vi "test Get Parameters.vi"(8 "error in":errorcluster, 11 "TestCase in":refnum<class "Scripting.lvclass">) -> (0 "error out":errorcluster, 3 "TestCase out":refnum<class "Scripting.lvclass">)   [LabVIEW 2020, in "Scripting.lvclass"]
uses:
  Scripting.lvclass
  <vilib>/addons/_JKI Toolkits/VI Tester/TestCase.llb/TestCase.lvclass
  Scripting/AIM/Constants.vi
  Scripting/AIM/AIM ARINC 429 Scripting.lvlib
  <vilib>/NI/NI VeriStand Encoding and Decoding/Encoding.ctl
  <vilib>/NI/NI VeriStand Encoding and Decoding/Encoding and Decoding.lvlib
  Shared/Parameter Definition.ctl
  <vilib>/NI VeriStand/Custom Device Tools/Custom Device Utility Library/Custom Device Utility Library.lvlib
  Shared/Label Properties.ctl
  <vilib>/NI VeriStand/Custom Device API/Custom Device API.lvlib
  Shared/Label.ctl
  Shared/Direction.ctl
  Shared/VS Channel Definition for Parameter.ctl
  Shared/Transfer Type.ctl
  Shared/VS Channels Definition for Label.ctl
  <vilib>/NI VeriStand/Custom Device Tools/Custom Device Utility Library/NI VeriStand - Search for Item by GUID.vi
  Shared/Transfer Speed.ctl
  C:/Program Files (x86)/National Instruments/LabVIEW 2020/vi.lib/addons/_JKI Toolkits/VI Tester/TestCase.llb/TestCase.lvclass
  C:/git/ni/niveristand-aim-arinc429-custom-device/Source/Custom Device Support/Tests/Unit/Scripting/Scripting.lvclass
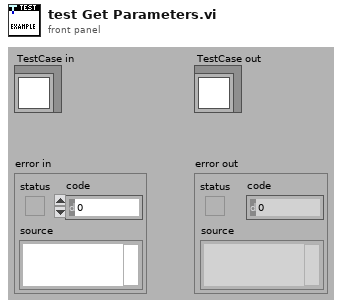
[diagram p1: front panel]
types:
  T1 = typedef "Transfer Speed.ctl" = enum16{"LO (12.5 kb/s)", "HI (100 kb/s)"}
  T2 = typedef "VS Channels Definition for Label.ctl" = cluster{"label (Dec)":u32, "parameters":T3[], "SDI value":u8, "SDI enabled":bool, "transfer type":T6, "create timestamp":bool, "transmit period":u32}
  T3 = typedef "VS Channel Definition for Parameter.ctl" = cluster{"name":string, "unit":string, "Parameter":T4}
  T4 = typedef "Parameter Definition.ctl" = cluster{"start index":i32, "size":i32, "encoding":T5, "signed":bool, "scale multiplier":dbl, "scale offset":dbl, "default value":dbl}
  T5 = typedef "Encoding and Decoding.lvlib/Encoding.ctl" = enum16{"BNR", "BCD", "Discrete"}
  T6 = typedef "Transfer Type.ctl" = enum16{"Scheduled", "Acyclic", "Block", "Strobe"}
  T7 = typedef "Direction.ctl" = enum16{"Rx", "Tx"}
  T8 = typedef "Label Properties.ctl" = cluster{"label (Dec)":T9, "SDI value":u8, "SDI enabled":bool}
  T9 = typedef "Label.ctl" = u8
  T10 = typedef "Custom Device API.lvlib/Custom Device Item Ref.ctl" = u64
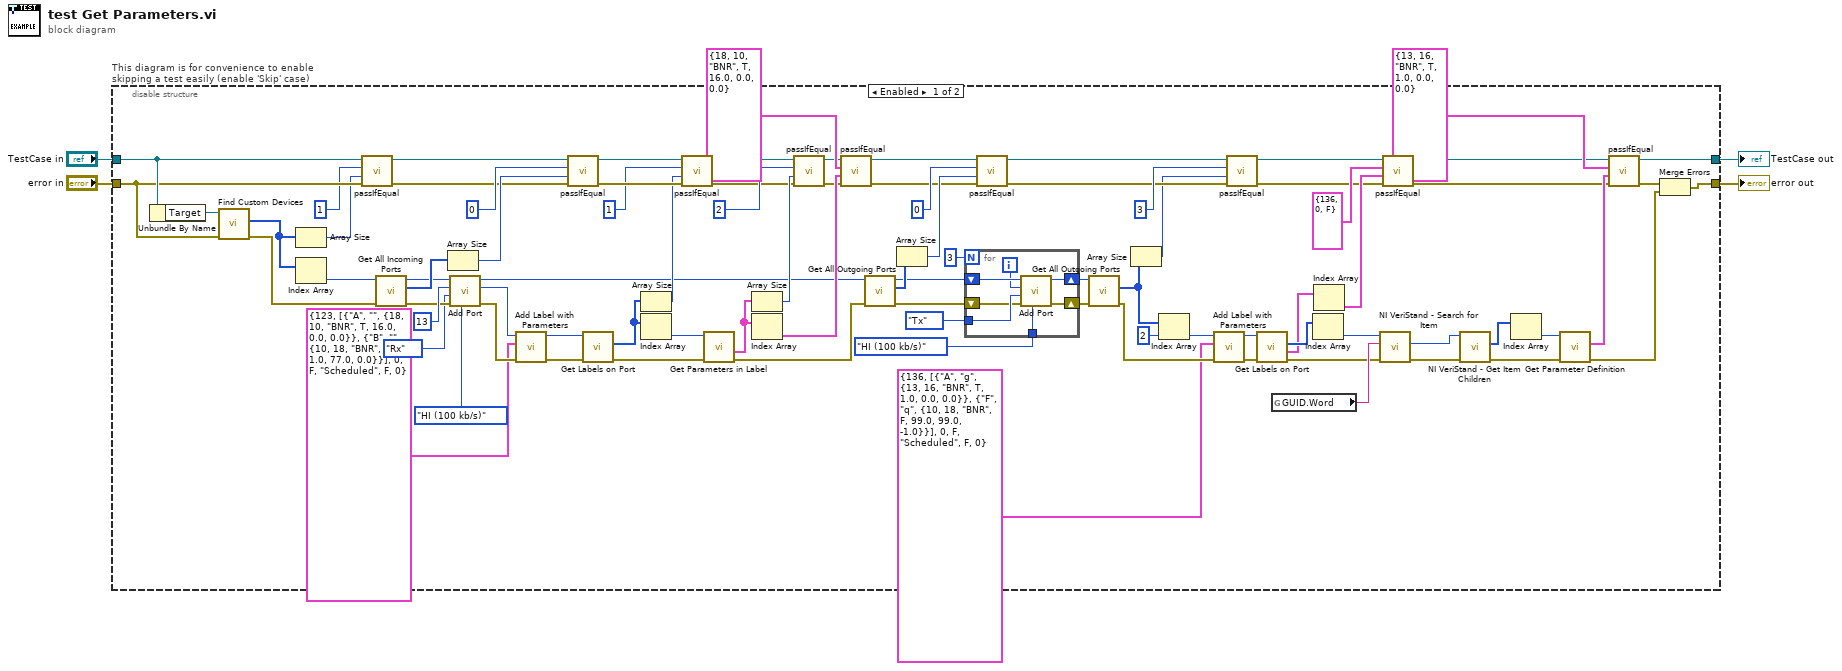
[diagram p0: block diagram]
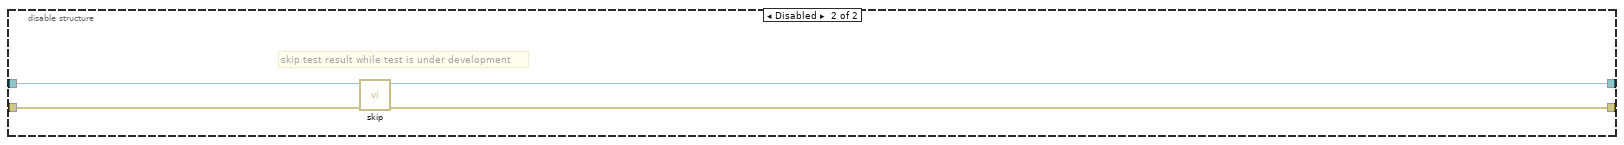
[diagram p2: hidden frame]
diagram:
  n1 = disable-structure "This diagram is for convenience to enable skipping a test easily (enable 'Skip' case)" shown="Enabled" {
    disable-tunnel: "TestCase in" -> [w87 w101]
    disable-tunnel: [w68 w99] -> w1
    disable-tunnel: [w70 w100] -> w3
    disable-tunnel: "error in" -> [w86 w98]
    frame Enabled {
      n2 = Unbundle By Name(w87) -> ("Target"=w89:refnum<k24>)
      n3 = call "Find Custom Devices.vi"("error in"=w86, "target in"=w89) -> ("error out"=w78:errorcluster, "AIM ARINC 429 custom devices"=w35:u64[])  [unwired: 7 in, 1 out]
      n4 = Array Size(array=w35) -> (size(s)=w84:i32)
      n5 = Index Array(array=w35) -> (element=w88:u64)  [unwired: 1 in]
      n6 = call-dynamic "passIfEqual.vi"("error in (no error)"=w86, "y"=w84, "x"=1 ("size(s)"), "TestCase in"=w87) -> ("error out"=w79:errorcluster, "TestCase out"=w80:refnum<class "Scripting.lvclass">)  [unwired: 6 in]
      n7 = call "Get All Incoming Ports.vi"("error in"=w78, "AIM ARINC 429 custom device in"=w88) -> ("error out"=w31:errorcluster, "incoming ports"=w83:T10[], "AIM ARINC 429 custom device out"=w34:T10)  [unwired: 7 in]
      n8 = Array Size(array=w83) -> (size(s)=w81:i32)
      n9 = call "Add Port.vi"("speed"=Transfer_Speed."HI (100 kb/s)", "error in"=w31, "direction"=Direction."Rx", "port number"=u16 13, "AIM ARINC 429 custom device in"=w34) -> ("error out"=w28:errorcluster, "port"=w29:T10, "AIM ARINC 429 custom device out"=w33:T10)  [unwired: 4 in]
      n10 = call "Add Label with Parameters.vi"("error in"=w28, "label"=T2 {"label (Dec)"=123, "parameters"=[{"name"="A", "unit"="", "Parameter"={"start index"=18, "size"=10, "encoding"=enum."BNR", "signed"=TRUE, "scale multiplier"=16.0, "scale offset"=0.0, "default value"=0.0}}, {"name"="B", "unit"="", "Parameter"={"start index"=10, "size"=18, "encoding"=enum."BNR", "signed"=FALSE, "scale multiplier"=1.0, "scale offset"=77.0, "default value"=0.0}}], "SDI value"=0, "SDI enabled"=FALSE, "transfer type"=enum."Scheduled", "create timestamp"=FALSE, "transmit period"=0}, "port ref"=w29) -> ("error out"=w25:errorcluster, "port ref out"=w26:T10)  [unwired: 7 in]
      n11 = call-dynamic "passIfEqual.vi"("error in (no error)"=w79, "y"=w81, "x"=0 ("size(s)"), "TestCase in"=w80) -> ("error out"=w62:errorcluster, "TestCase out"=w63:refnum<class "Scripting.lvclass">)  [unwired: 6 in]
      n12 = call "Get Labels on Port.vi"("error in"=w25, "port in"=w26) -> ("error out"=w50:errorcluster, "labels"=w51:T10[])  [unwired: 6 in, 2 out]
      n13 = Array Size(array=w51) -> (size(s)=w59:i32)
      n14 = Index Array(array=w51) -> (element=w61:T10)  [unwired: 1 in]
      n15 = call-dynamic "passIfEqual.vi"("error in (no error)"=w62, "y"=w59, "x"=1 ("size(s)"), "TestCase in"=w63) -> ("error out"=w54:errorcluster, "TestCase out"=w55:refnum<class "Scripting.lvclass">)  [unwired: 6 in]
      n16 = call "Get Parameters in Label.vi"("error in"=w50, "label in"=w61) -> ("error out"=w65:errorcluster, "parameter definitions"=w58:T4[])  [unwired: 6 in, 2 out]
      n17 = Array Size(array=w58) -> (size(s)=w56:i32)
      n18 = Index Array(array=w58) -> (element=w64:T4)  [unwired: 1 in]
      n19 = call-dynamic "passIfEqual.vi"("error in (no error)"=w54, "y"=w56, "x"=2 ("size(s)"), "TestCase in"=w55) -> ("error out"=w52:errorcluster, "TestCase out"=w53:refnum<class "Scripting.lvclass">)  [unwired: 6 in]
      n20 = call-dynamic "passIfEqual.vi"("error in (no error)"=w52, "y"=w64, "x"=T4 {"start index"=18, "size"=10, "encoding"=enum."BNR", "signed"=TRUE, "scale multiplier"=16.0, "scale offset"=0.0, "default value"=0.0} ("parameter definition"), "TestCase in"=w53) -> ("error out"=w74:errorcluster, "TestCase out"=w75:refnum<class "Scripting.lvclass">)  [unwired: 6 in]
      n21 = call "Get All Outgoing Ports.vi"("error in"=w65, "AIM ARINC 429 custom device in"=w33) -> ("error out"=w22:errorcluster, "outgoing ports"=w73:T10[], "AIM ARINC 429 custom device out"=w24:T10)  [unwired: 7 in]
      n22 = Array Size(array=w73) -> (size(s)=w76:i32)
      n23 = for {
        N: 3 -> [_]
        tunnel: Direction."Tx" ("direction") -> [w95]
        shift-right: [w93] -> w21
        shift-left: w22 -> [w94]
        shift-right: [w92] -> w20
        shift-left: w24 -> [w97]
        tunnel: Transfer_Speed."HI (100 kb/s)" ("speed") -> [w91]
        i -> [w96]
        n24 = call "Add Port.vi"("speed"=w91, "error in"=w94, "direction"=w95, "port number"=w96, "AIM ARINC 429 custom device in"=w97) -> ("error out"=w93:errorcluster, "AIM ARINC 429 custom device out"=w92:T10)  [unwired: 4 in, 1 out]
      }
      n25 = call-dynamic "passIfEqual.vi"("error in (no error)"=w74, "y"=w76, "x"=0 ("size(s)"), "TestCase in"=w75) -> ("error out"=w17:errorcluster, "TestCase out"=w16:refnum<class "Scripting.lvclass">)  [unwired: 6 in]
      n26 = call "Get All Outgoing Ports.vi"("error in"=w21, "AIM ARINC 429 custom device in"=w20) -> ("error out"=w9:errorcluster, "outgoing ports"=w15:T10[])  [unwired: 7 in, 1 out]
      n27 = Array Size(array=w15) -> (size(s)=w14:i32)
      n28 = Index Array(array=w15, index=2) -> (element=w11:T10)
      n29 = call "Add Label with Parameters.vi"("error in"=w9, "label"=T2 {"label (Dec)"=136, "parameters"=[{"name"="A", "unit"="g", "Parameter"={"start index"=13, "size"=16, "encoding"=enum."BNR", "signed"=TRUE, "scale multiplier"=1.0, "scale offset"=0.0, "default value"=0.0}}, {"name"="F", "unit"="q", "Parameter"={"start index"=10, "size"=18, "encoding"=enum."BNR", "signed"=FALSE, "scale multiplier"=99.0, "scale offset"=99.0, "default value"=-1.0}}], "SDI value"=0, "SDI enabled"=FALSE, "transfer type"=enum."Scheduled", "create timestamp"=FALSE, "transmit period"=0}, "port ref"=w11) -> ("error out"=w8:errorcluster, "port ref out"=w10:T10)  [unwired: 7 in]
      n30 = call-dynamic "passIfEqual.vi"("error in (no error)"=w17, "y"=w14, "x"=3 ("size(s)"), "TestCase in"=w16) -> ("error out"=w13:errorcluster, "TestCase out"=w12:refnum<class "Scripting.lvclass">)  [unwired: 6 in]
      n31 = call "Get Labels on Port.vi"("error in"=w8, "port in"=w10) -> ("error out"=w46:errorcluster, "labels properties"=w43:T8[], "labels"=w49:T10[])  [unwired: 6 in, 1 out]
      n32 = global read "Constants.vi" "GUID.Word"() -> (w47:string)
      n33 = Index Array(array=w49) -> (element=w48:T10)  [unwired: 1 in]
      n34 = Index Array(array=w43) -> (element=w42:T8)  [unwired: 1 in]
      n35 = call-poly <vilib>:"NI VeriStand - Search for Item.vi"("error in"=w46, "Item GUID"=w47, "Section Ref in"=w48) -> ("error out"=w39:errorcluster, "Item Ref"=w40:T10)  [unwired: 5 in, 2 out]
      n36 = call-dynamic "passIfEqual.vi"("error in (no error)"=w13, "y"=w42, "x"=T8 {"label (Dec)"=136, "SDI value"=0, "SDI enabled"=FALSE} ("element"), "TestCase in"=w12) -> ("error out"=w44:errorcluster, "TestCase out"=w45:refnum<class "Scripting.lvclass">)  [unwired: 6 in]
      n37 = call <vilib>:"NI VeriStand - Get Item Children.vi"("error in (no error)"=w39, "Item Ref in"=w40) -> ("error out"=w38:errorcluster, "Child Refs"=w36:T10[])  [unwired: 6 in, 2 out]
      n38 = Index Array(array=w36) -> (element=w37:T10)  [unwired: 1 in]
      n39 = call "Get Parameter Definition.vi"("error in"=w38, "parameter ref in"=w37) -> ("error out"=w71:errorcluster, "parameter definition"=w69:T4)  [unwired: 7 in, 1 out]
      n40 = call-dynamic "passIfEqual.vi"("error in (no error)"=w44, "y"=w69, "x"=T4 {"start index"=13, "size"=16, "encoding"=enum."BNR", "signed"=TRUE, "scale multiplier"=1.0, "scale offset"=0.0, "default value"=0.0} ("parameter definition"), "TestCase in"=w45) -> ("error out"=w67:errorcluster, "TestCase out"=w68:refnum<class "Scripting.lvclass">)  [unwired: 6 in]
      n41 = Merge Errors(w67, w71) -> (w70:errorcluster)
    }
    frame Disabled {
      # "skip test result while test is under development"
      n42 = call <vilib>:"skip.vi"("error in (no error)"=w98, "TestCase in"=w101) -> ("error out"=w100:errorcluster, "TestCase out"=w99:refnum<class "Scripting.lvclass">)  [unwired: 8 in]
    }
  }
  "error out" <- w3
  "TestCase out" <- w1
